vi "PuT3 TCP Austausch.vi"(8 "error in":errorcluster, 11 "Anfrage":string) -> (0 "error out":errorcluster, 3 "Antwort":string)   [LabVIEW 2026]
doc: "Eine Anfrage an die lokale Steckwerkbank. Antwort: Status und Messdaten als tabulatorgetrennte Zahlen."
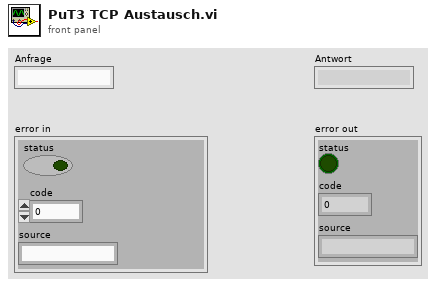
[diagram p1: front panel]
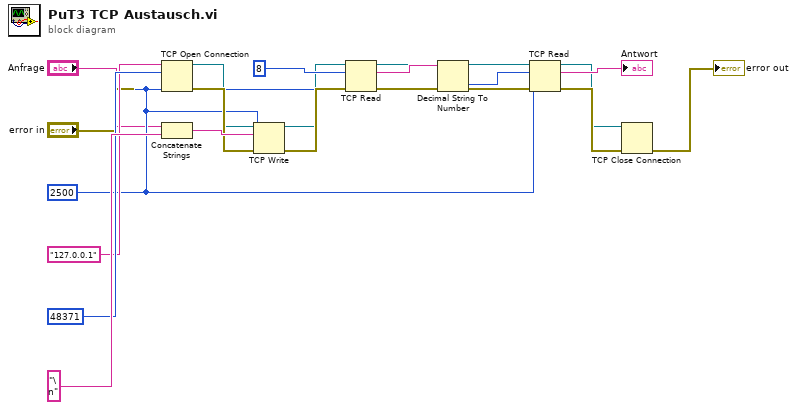
[diagram p0: block diagram]
diagram:
  w3 = 2500
  n1 = TCP Open Connection(address="127.0.0.1", remote port or service name=u16 48371, timeout ms (60000)=w3, error in (no error)="error in") -> (connection ID=w6:refnum<k5>, error out=w7:errorcluster)  [unwired: 1 in]
  n2 = Concatenate Strings("Anfrage", "\n") -> (w9:string)
  n3 = TCP Write(connection ID=w6, data in=w9, error in (no error)=w7, 9:w3) -> (connection ID out=w10:refnum<k5>, error out=w11:errorcluster)  [unwired: 1 out]
  n4 = TCP Read(connection ID=w10, bytes to read=8, error in (no error)=w11, 9:w3) -> (connection ID out=w13:refnum<k5>, data out=w14:string, error out=w15:errorcluster)  [unwired: 1 in]
  n5 = Decimal String To Number(string=w14) -> (number=w16:i32)  [unwired: 2 in, 1 out]
  n6 = TCP Read(connection ID=w13, bytes to read=w16, error in (no error)=w15, 9:w3) -> (connection ID out=w17:refnum<k5>, data out=→"Antwort":string, error out=w19:errorcluster)  [unwired: 1 in]
  n7 = TCP Close Connection(connection ID=w17, error in (no error)=w19) -> (error out=→"error out":errorcluster)  [unwired: 1 in, 1 out]
